vi "VIH UI - Undo Focused Control - Keyboard Hit.vi"(8 "FocusObj":refnum<vi>, 9 "PlatMods":cluster{"Shift":bool, "Ctrl":bool, "Alt":bool}, 10 "VKey":T1, 11 "Char":i16) -> (0 "Discard":bool)   [LabVIEW 2014]
doc: "::: VI Helpeks :::\nCopyright (c) 2000-2026 Konstantin Shifershteyn. All rights reserved."
uses:
  <vilib>/event_ctls.llb/eventvkey.ctl
panel:
  # "VI Helpeks\nCopyright (c) 2012-2026 Konstantin Shifershteyn"
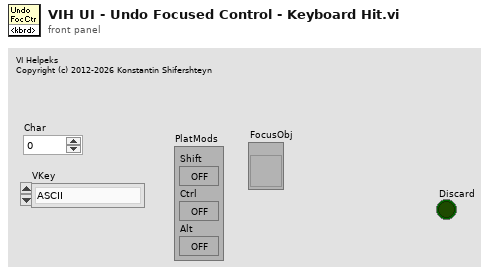
[diagram p1: front panel]
types:
  T1 = typedef "eventvkey.ctl" = enum16{"ASCII", "Enter", "Return", "Shift", "Ctrl", "Alt", "Cmd", "Opt", "Caps", "NumLock", "Clear", "Break", "Up", "Down", "Left", "Right", "Insert", "Delete", "Home", "End", "PageUp", "PageDown", "Escape", "Help", "Pause", "ScrollLock", "F1", "F2", "F3", "F4", "F5", "F6", "F7", "F8", "F9", "F10", "F11", "F12", "F13", "F14", "F15", "F16", "F17", "F18", "F19", "F20", "F21", "F22", "F23", "F24", "Play", "VolumeUp", "VolumeDown", "Mute", "Two Byte Char"}
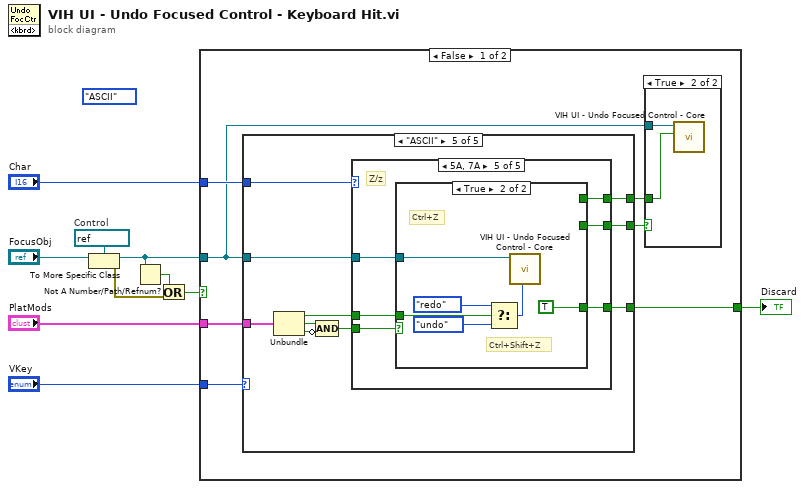
[diagram p0: block diagram]
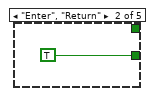
[diagram p4: hidden frame]
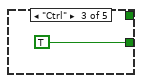
[diagram p5: hidden frame]
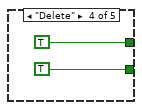
[diagram p6: hidden frame]
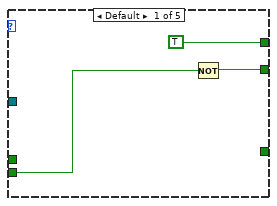
[diagram p7: hidden frame]
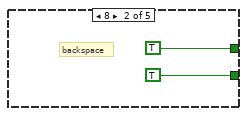
[diagram p8: hidden frame]
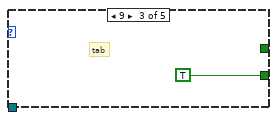
[diagram p9: hidden frame]
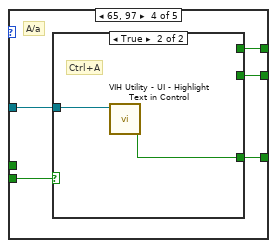
[diagram p10: hidden frame]
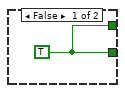
[diagram p11: hidden frame]
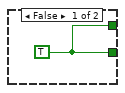
[diagram p12: hidden frame]
diagram:
  w6 = refnum<vi> refnum  # Control
  (unwired) eventvkey."ASCII" ("VKey")
  n1 = To More Specific Class(target class=w6, reference="FocusObj") -> (specific class reference=w4:refnum<vi>, error out=w2:errorcluster)  [unwired: 1 in]
  n2 = Not A Number/Path/Refnum?(number/path/refnum=w4) -> (NaN/Path/Refnum?=w3:bool)
  n3 = Or(x=w3, y=w2) -> (x .or. y?=w1:bool)
  n4 = case shown="False" w1 {
    tunnel: "Char" -> [w16 _]
    tunnel: "VKey" -> [w15 _]
    tunnel: "PlatMods" -> [w14 _]
    tunnel: [w13 _] -> w7
    tunnel: w4 -> [w12 _]
    frame False {
      n5 = case shown="\"ASCII\"" w15 {
        tunnel: w16 -> [_ _ _ _ w33]
        tunnel: w14 -> [_ _ _ _ w32]
        tunnel: w12 -> [_ _ _ _ w28]
        tunnel: [_ _ _ _ w27] -> w13
        tunnel: [_ TRUE TRUE TRUE w25] -> w17
        tunnel: [_ _ _ TRUE w24] -> w11
        frame Default {
        }
        frame "Enter", "Return" {
        }
        frame "Ctrl" {
        }
        frame "Delete" {
        }
        frame "ASCII" {
          n6 = Unbundle(w32) -> ("Shift"=w26:bool, "Ctrl"=w31:bool, "Alt"=w30:bool)
          n7 = Compound Arithmetic op=AND(w31, invert w30) -> (w29:bool)
          n8 = case shown="5A, 7A" w33 {
            tunnel: w29 -> [w35 _ _ w44 w53]
            tunnel: w28 -> [_ _ _ w43 w52]
            tunnel: [_ _ _ w42 w51] -> w27
            tunnel: w26 -> [_ _ _ _ w50]
            tunnel: [w34 TRUE TRUE w41 w49] -> w25
            tunnel: [TRUE TRUE _ w40 w48] -> w24
            frame Default {
              n9 = Not(x=w35) -> (.not. x?=w34:bool)
            }
            frame 8 {
              # "backspace"
            }
            frame 9 {
              # "tab"
            }
            frame 65, 97 {
              # "A/a"
              n10 = case shown="True" w44 {
                tunnel: w43 -> [_ w47]
                tunnel: [_ w46] -> w42
                tunnel: [w45 _] -> w41
                tunnel: [w45 _] -> w40
                frame False {
                  w45 = TRUE
                }
                frame True {
                  # "Ctrl+A"
                  n11 = call "VIH Utility - UI - Highlight Text in Control.vi"("FocusObj"=w47) -> ("OK"=w46:bool)  [unwired: 10 in]
                }
              }
            }
            frame 90, 122 {
              # "Z/z"
              n12 = case shown="True" w53 {
                tunnel: w52 -> [_ w58]
                tunnel: [_ TRUE] -> w51
                tunnel: w50 -> [_ w60]
                tunnel: [w54 _] -> w49
                tunnel: [w54 _] -> w48
                frame False {
                  w54 = TRUE
                }
                frame True {
                  # "Ctrl+Shift+Z"
                  # "Ctrl+Z"
                  n13 = Select(t=enum16{"Init", "status", "save", "undo", "redo"}."redo" ("cmd (click)"), s=w60, f=enum16{"Init", "status", "save", "undo", "redo"}."undo" ("cmd (click)")) -> (s? t:f=w59:enum16{"Init", "status", "save", "undo", "redo"})
                  n14 = call "VIH UI - Undo Focused Control - Core.vi"("cmd (save)"=w59, "Ctl Refnum"=w58) -> ()  [unwired: 7 in, 3 out]
                }
              }
            }
          }
        }
      }
      n15 = case shown="True" w17 {
        tunnel: w12 -> [_ w19]
        tunnel: w11 -> [_ w18]
        frame False {
        }
        frame True {
          n16 = call "VIH UI - Undo Focused Control - Core.vi"("Need Selection (F)"=w18, "Ctl Refnum"=w19) -> ()  [unwired: 7 in, 3 out]
        }
      }
    }
    frame True {
    }
  }
  "Discard" <- w7
